vi "Write protocol.vi"(8 "error in (no error)":errorcluster, 10 "ZM-CP-communication_protocol.lvlib:ZM-CP-communication_protocol.lvclass":refnum<class "ZM-CP-communication_protocol.lvclass">, 11 "ZM-CM-communication_manager in":refnum<class "ZM-CM-communication_manager.lvclass">) -> (0 "error out":errorcluster, 3 "ZM-CM-communication_manager out":refnum<class "ZM-CM-communication_manager.lvclass">)   [LabVIEW 2020, in "ZM-CM-communication_manager.lvlib" / "ZM-CM-communication_manager.lvclass"]
doc: "Writes one field of this class's private data. Generated by lvai_create_accessors from the class private data control."
uses:
  ZM-CM-communication_manager.lvclass
  protocol/ZM-CP-communication_protocol/ZM-CP-communication_protocol/ZM-CP-communication_protocol.lvclass
  ZM-CM-communication_manager.lvclass/ZM-CM-communication_manager.ctl
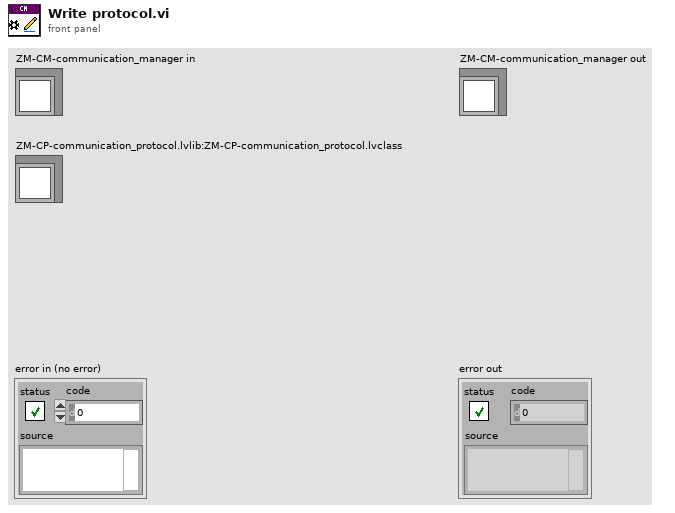
[diagram p1: front panel]
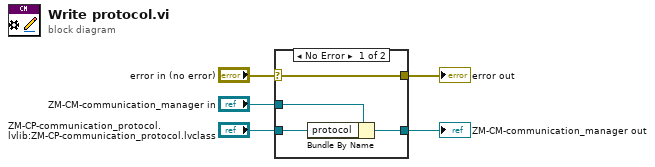
[diagram p0: block diagram]
diagram:
  n1 = case shown="No Error" "error in (no error)" {
    selector: "error in (no error)" -> [w9 w10]
    tunnel: [w9 w10] -> w4
    tunnel: [w7 w11] -> w2
    tunnel: "ZM-CM-communication_manager in" -> [w8 w11]
    tunnel: "ZM-CP-communication_protocol.lvlib:ZM-CP-communication_protocol.lvclass" -> [w6 _]
    frame No Error {
      n2 = Bundle By Name(cluster=w8, "protocol"=w6) -> (w7:refnum<class "ZM-CM-communication_manager.lvclass">)
    }
    frame Error {
    }
  }
  "error out" <- w4
  "ZM-CM-communication_manager out" <- w2
